vi "user32 GetClassNameW.vi"(0 "hWnd":u64, 5 "nMaxCount":i32=256, 11 "error in":errorcluster) -> (4 "class name":string, 6 "return value":i32, 15 "error out":errorcluster)   [LabVIEW 2020, in "RemoteVI.lvlib"]
doc: "Returns the class name of the window hWnd through user32.dll GetClassNameW (stdcall, called in any thread), e.g. LVMenuWnd for a LabVIEW ring menu. The buffer is nMaxCount UTF-16 code units of zeros, and the name is cut at its terminating 0 and narrowed code unit by code unit to bytes - exact for ASCII class names, which is what window classes are in practice. return value is the number of characters copied, 0 on failure. When error in carries an error the DLL is not called. Generated by scripts\\Build Win32 Wrappers.vi - do not edit by hand, rebuild it."
uses:
  RemoteVI.lvlib
  user32.dll
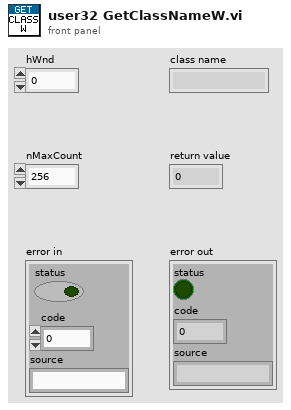
[diagram p1: front panel]
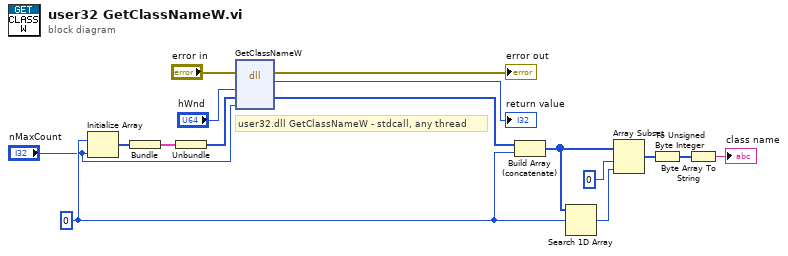
[diagram p0: block diagram]
diagram:
  w9 = u16 0
  # "user32.dll GetClassNameW - stdcall, any thread"
  n1 = Initialize Array(w9, "nMaxCount") -> (w10:u16[])
  n2 = Bundle(w10) -> (w11:cluster{u16[]})  [unwired: 1 in]
  n3 = Unbundle(w11) -> (w2:u16[])
  n4 = dll-call lib="user32.dll" fn="GetClassNameW"(error in="error in", "hWnd"="hWnd", "lpClassName"=w2, "nMaxCount"="nMaxCount") -> (error out=→"error out":errorcluster, →"return value":i32, "lpClassName"=w1:u16[])  [unwired: 4 in, 1 out]
  n5 = Build Array (concatenate)(w1, w9) -> (w12:u16[])
  n6 = Search 1D Array(1D array=w12, element=w9) -> (index of element=w13:i32)  [unwired: 1 in]
  n7 = Array Subset(array=w12, index=0, length=w13) -> (w15:u16[])
  n8 = To Unsigned Byte Integer(number=w15) -> (unsigned 8bit integer=w16:u8[])
  n9 = Byte Array To String(unsigned byte array=w16) -> (string=→"class name":string)
